vi "UI.vi"(8 "error in (no error)":errorcluster, 11 "View in":refnum<class "View.lvclass">) -> (0 "error out":errorcluster, 3 "View out":refnum<class "View.lvclass">)   [LabVIEW 2024, in "Page2.lvlib" / "View.lvclass"]
uses:
  View.lvclass
  View.lvclass/View.ctl
  NavigatableView/NavigatableView.lvclass
panel:
  in  "GoToPage1Button":bool
  in  "PreviousPageButton":bool
  in  "NextPageButton":bool
  # "Page 2"
  # "<- Go clears the navigation stack and pushes a\n     specified page onto the empty stack."
  # "<- Push pushes a specified page onto the end of\n     an existing stack."
  # "<- Pop removes the last page from the stack."
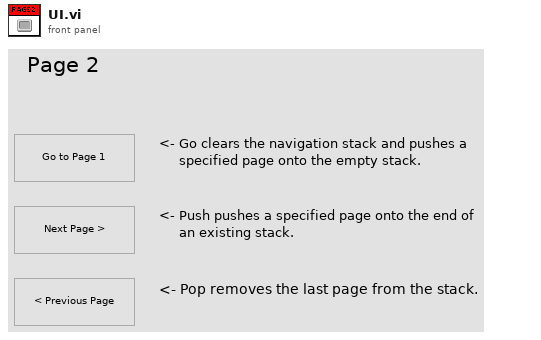
[diagram p1: front panel]
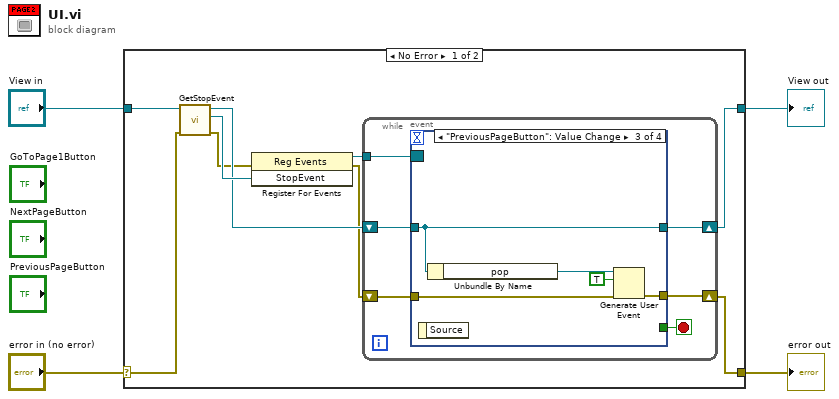
[diagram p0: block diagram]
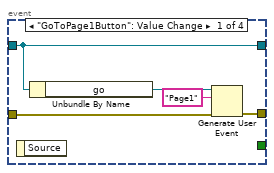
[diagram p2: hidden frame]
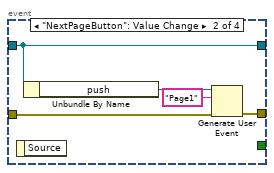
[diagram p3: hidden frame]
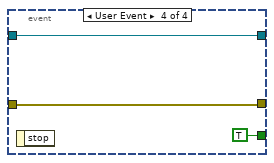
[diagram p4: hidden frame]
diagram:
  n1 = case shown="No Error" "error in (no error)" {
    selector: "error in (no error)" -> [w12 w39]
    tunnel: [w5 w39] -> w2
    tunnel: [w8 w38] -> w3
    tunnel: "View in" -> [w13 w38]
    frame No Error {
      n2 = call "GetStopEvent.vi"("error in (no error)"=w12, "NavigatableView in"=w13) -> ("error out"=w6:errorcluster, "StopEvent"=w10:refnum<user-event>, "NavigatableView out"=w9:refnum<class "View.lvclass">)  [unwired: 7 in]
      n3 = register-events(error in=w6, w10) -> (reference out=w11:refnum<event-registration>, error out=w7:errorcluster)  [unwired: 1 in]
      n4 = while {
        tunnel: w11 -> [w19]
        shift-right: [w16] -> w8
        shift-left: w9 -> [w17]
        shift-right: [w15] -> w5
        shift-left: w7 -> [w14]
        stop <- w18 stop-if-true
        n5 = event shown="[2] \"PreviousPageButton\": Value Change" {
          selector: w19 -> [_ _ _ _]
          dyn-events: _ -> [_ _ _ _]
          timeout: _ -> [_ _ _ _]
          tunnel: [_ _ _ TRUE] -> w18
          tunnel: w17 -> [w22 w27 w33 w36]
          tunnel: [w22 w27 w33 w36] -> w16
          tunnel: [w21 w25 w30 w35] -> w15
          tunnel: w14 -> [w20 w26 w31 w35]
          event "GoToPage1Button": Value Change {
            n6 = event-data() -> ()  [unwired: 1 in, 1 out]
            n7 = Unbundle By Name(w22) -> ("go"=w24:refnum<user-event>)
            n8 = Generate User Event(user event=w24, event data cluster="Page1" ("event data"), error in=w20) -> (error out=w21:errorcluster)  [unwired: 1 in, 1 out]
          }
          event "NextPageButton": Value Change {
            n9 = event-data() -> ()  [unwired: 1 in, 1 out]
            n10 = Unbundle By Name(w27) -> ("push"=w29:refnum<user-event>)
            n11 = Generate User Event(user event=w29, event data cluster="Page1" ("event data"), error in=w26) -> (error out=w25:errorcluster)  [unwired: 1 in, 1 out]
          }
          event "PreviousPageButton": Value Change {
            n12 = event-data() -> ()  [unwired: 1 in, 1 out]
            n13 = Unbundle By Name(w33) -> ("pop"=w34:refnum<user-event>)
            n14 = Generate User Event(user event=w34, event data cluster=TRUE ("event data"), error in=w31) -> (error out=w30:errorcluster)  [unwired: 1 in, 1 out]
          }
          event User Event {
            n15 = event-data() -> ()  [unwired: 1 in, 1 out]
          }
        }
      }
    }
    frame Error {
    }
  }
  "error out" <- w2
  "View out" <- w3
